vi "Get Lines from String.vi"(8 "error in (no error)":errorcluster, 11 "Dialog in":refnum<class "Dialog.lvclass">) -> (0 "error out":errorcluster, 1 "Lines":string[](array[string]), 2 "# lines":i32, 3 "Dialog out":refnum<class "Dialog.lvclass">)   [LabVIEW 2012, in "Dialog.lvlib" / "Dialog.lvclass"]
uses:
  Dialog.lvclass
  Dialog.lvclass/Dialog.ctl
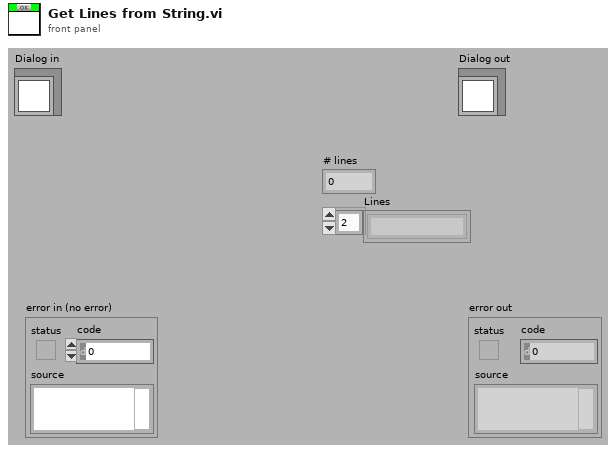
[diagram p1: front panel]
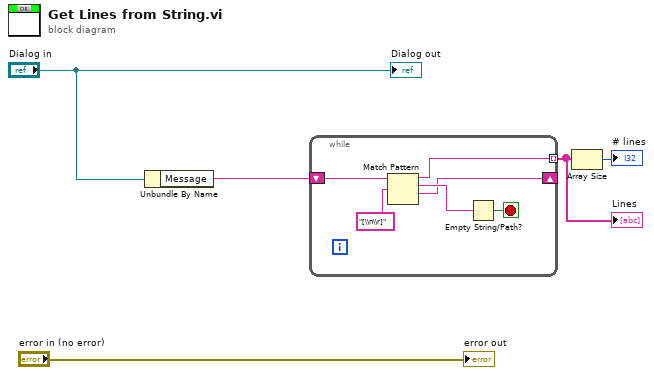
[diagram p0: block diagram]
diagram:
  n1 = Unbundle By Name("Dialog in") -> ("Message"=w1:string)
  n2 = while {
    tunnel: [w9] -> w5 mode=indexing
    shift-right: [w6] -> _
    shift-left: w1 -> [w10]
    stop <- w11 stop-if-true
    n3 = Match Pattern(string=w10, regular expression="[\\n\\r]") -> (before substring=w9:string, match substring=w7:string, after substring=w6:string)  [unwired: 2 out]
    n4 = Empty String/Path?(string/path=w7) -> (empty?=w11:bool)
  }
  "Lines" <- w5
  n5 = Array Size(array=w5) -> (size(s)=→"# lines":i32)
  "Dialog out" <- "Dialog in"
  "error out" <- "error in (no error)"
